vi "Measure.vi"(8 "error in (no error)":errorcluster, 9 "measurement configuration":variant, 10 "measure call context in":refnum<class "Measure Call Context.lvclass">, 11 "measurement plugin in":refnum<class "Automotive Ethernet Frame Generator.lvclass">) -> (0 "error out":errorcluster, 1 "measurement results":variant, 2 "measure call context out":refnum<class "Measure Call Context.lvclass">, 3 "measurement plugin out":refnum<class "Automotive Ethernet Frame Generator.lvclass">)   [LabVIEW 2025, in "Automotive Ethernet Frame Generator.lvclass"]
uses:
  Automotive Ethernet Frame Generator.lvclass
  Automotive Ethernet Frame Generator.lvclass/Automotive Ethernet Frame Generator.ctl
  Measurement Configuration.ctl
  OOB gRPC Server/OOB gRPC Server.lvlib
  OOB Data Transfer/OOB Data Transfer.lvlib
  <vilib>/Plug-In SDKs/Measurements/Measure Call Context/Measure Call Context.lvclass
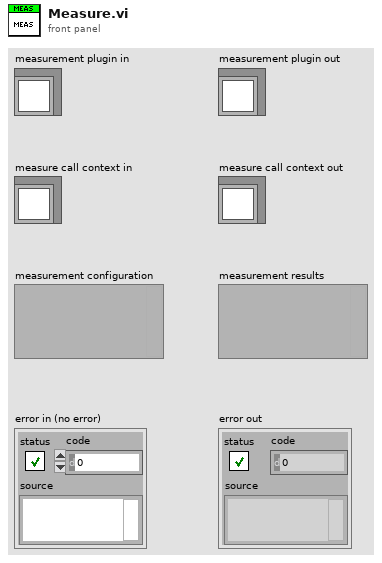
[diagram p1: front panel]
types:
  T1 = typedef "Automotive Ethernet Frame Generator.lvclass/Measurement Configuration.ctl" = cluster{"INTERFACE NAME STRING":string, "Payload":string, "Protocol Layer 2":cluster{"Has VLAN":bool, "VLAN TAG":cluster{"TPID":u16, "PRIORITY":u8, "DEI":bool, "VID":u16}, "DESTINATION MAC ADDRESS":string, "ETHERTYPE":u16}, "SEND FRAME":bool, "CYCLE?":bool}
  T2 = typedef "Automotive Ethernet Frame Generator.lvclass/Measurement Results.ctl" = cluster{"Transmitting":bool, "RECEIVED PACKETS":i32, "STATUS":string, "OOB gRPC Port":i32}
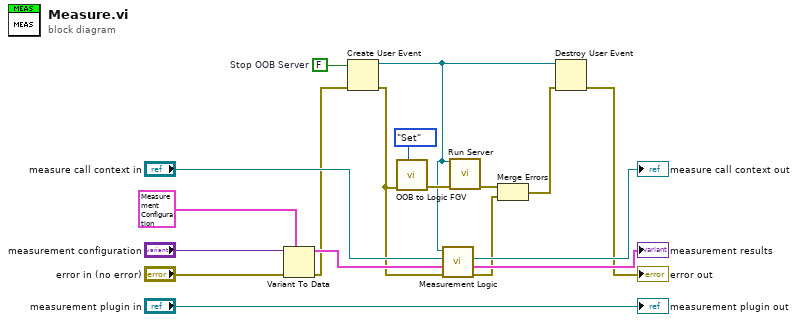
[diagram p0: block diagram]
diagram:
  w10 = FALSE  # Stop OOB Server
  n1 = Variant To Data(error in="error in (no error)", type=T1 {"INTERFACE NAME STRING"="Lorem ipsum dolor sit", "Payload"="", "Protocol Layer 2"={"Has VLAN"=FALSE, "VLAN TAG"={"TPID"=0, "PRIORITY"=0, "DEI"=FALSE, "VID"=0}, "DESTINATION MAC ADDRESS"="", "ETHERTYPE"=0}, "SEND FRAME"=TRUE, "CYCLE?"=FALSE} ("measurement configuration"), Variant="measurement configuration") -> (data=w11:T1, error out=w9:errorcluster)
  n2 = Create User Event(user event datatype=w10, error in=w9) -> (user event=w1:refnum<user-event>, error out=w8:errorcluster)
  n3 = call "OOB to Logic FGV.vi"("Op (Get)"=enum16{"Get", "Set"}."Set", "error in (no error)"=w8) -> ("error out"=w3:errorcluster)  [unwired: 8 in, 1 out]
  n4 = call "Measurement Logic.vi"("error in"=w8, "measurement configuration"=w11, "measure call context in"="measure call context in", "user event out"=w1) -> ("error out"=w5:errorcluster, "measurement results"=→"measurement results":T2, "measure call context out"=→"measure call context out":refnum<class "Measure Call Context.lvclass">)  [unwired: 5 in]
  n5 = call "Run Server.vi"("error in (no error)"=w3, "Stop OOB Server UE"=w1) -> ("error out"=w2:errorcluster)  [unwired: 9 in]
  n6 = Merge Errors(w2, w5) -> (w6:errorcluster)
  n7 = Destroy User Event(user event=w1, error in=w6) -> (error out=→"error out":errorcluster)
  "measurement plugin out" <- "measurement plugin in"
